vi "B folder set parameter.vi"(11 "folder list":string[](array[string])) -> (3 "S array":T1(array[cluster]))   [LabVIEW 2018]
panel:
  out "逆文字列":string
  out "Folder Namte":string
  out "list#":i32=3
  out "数値":i32
  in  "S New Info and MiN out":T2={"Sample Sequence"="GATGATGATGATGATGAT", "Right Read MIN"=6, "Filter P"=0, "STD Type"=enum."Region", "Base Table"=[], "Selection"=enum."10kHz", "noise MAX"=3, "Sample name"=""} {"Base Table"."Value 3" format="%.2g"}
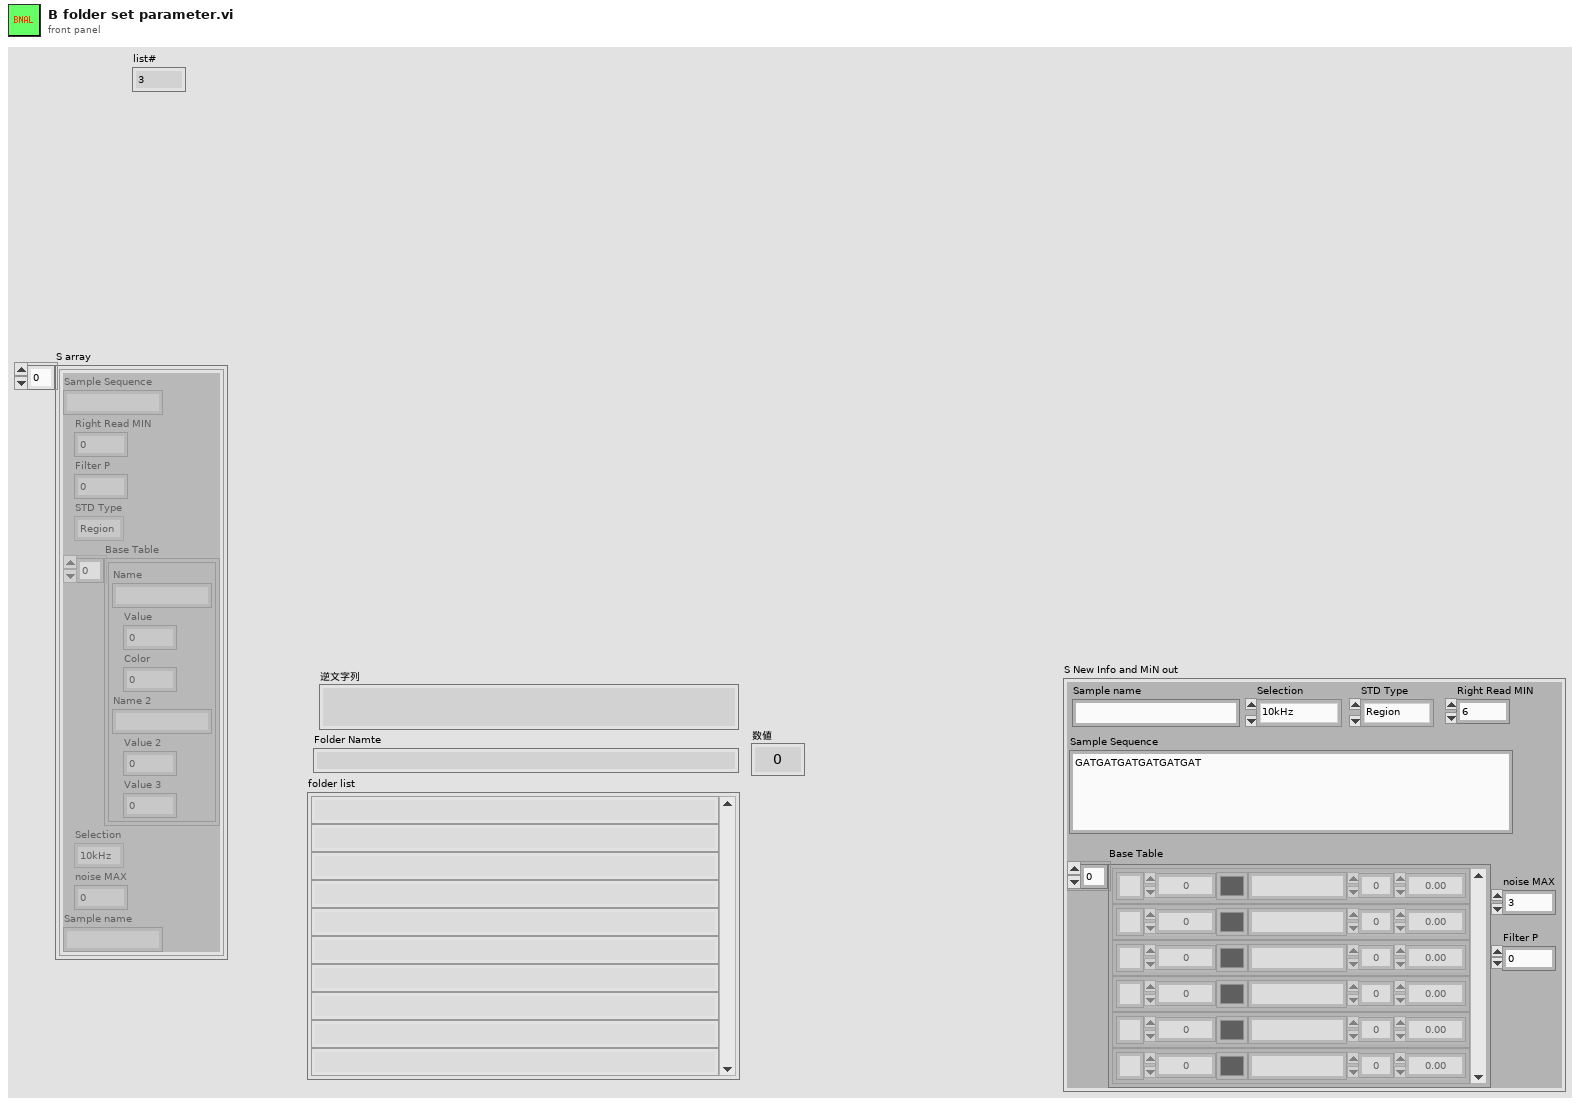
[diagram p1: front panel]
types:
  T1 = cluster{"Sample Sequence":string, "Right Read MIN":i32, "Filter P":i32, "STD Type":enum16{"Region", "Each", "Fixed"}, "Base Table":cluster{"Name":string, "Value":dbl, "Color":u32, "Name 2":string, "Value 2":dbl, "Value 3":dbl}[], "Selection":enum16{"10kHz", "100kHz"}, "noise MAX":i32, "Sample name":string}[]
  T2 = cluster{"Sample Sequence":string, "Right Read MIN":i32, "Filter P":i32, "STD Type":enum16{"Region", "Each", "Fixed"}, "Base Table":cluster{"Name":string, "Value":dbl, "Color":u32, "Name 2":string, "Value 2":dbl, "Value 3":dbl}[], "Selection":enum16{"10kHz", "100kHz"}, "noise MAX":i32, "Sample name":string}
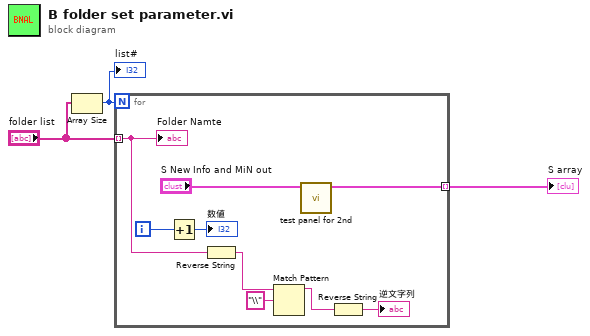
[diagram p0: block diagram]
diagram:
  n1 = Array Size(array="folder list") -> (size(s)=w1:i32)
  "list#" <- w1
  n2 = for {
    N: w1 -> [_]
    tunnel: [w11] -> w3 mode=indexing
    tunnel: "folder list" -> [w4] mode=indexing
    i -> [w10]
    n3 = Increment(x=w10) -> (x+1=→"数値":i32)
    n4 = Reverse String(1:w4) -> (0:w6:string)
    n5 = Match Pattern(string=w6, regular expression="\\" ("正規表現")) -> (before substring=w8:string)  [unwired: 1 in, 3 out]
    n6 = call "test panel for 2nd.vi"("S New Info and MiN"="S New Info and MiN out") -> ("S New Info and MiN out"=w11:T2)  [unwired: 8 in, 2 out]
    n7 = Reverse String(1:w8) -> (0:→"逆文字列":string)
    "Folder Namte" <- w4
  }
  "S array" <- w3
